vi "SMO.jsonRPC.SendAsyncRequest.vi"(7 "Notification":bool, 8 "error in (no error)":errorcluster, 9 "Parameters":variant, 10 "Method":string, 11 "SMO.jsonRPC in":refnum<class "SMO.jsonRPC.lvclass">) -> (0 "error out":errorcluster, 2 "id":i32, 3 "SMO.jsonRPC out":refnum<class "SMO.jsonRPC.lvclass">)   [LabVIEW 2013, in "SMO.jsonRPC.lvclass"]
uses:
  SMO.jsonRPC.lvclass
  Typedefs/Request--Cluster.ctl
  <vilib>/JKI/JKI JSON RPC Specification/Request/Request.lvclass
  <vilib>/JKI/JKI JSON RPC Specification/Response/Response.lvclass
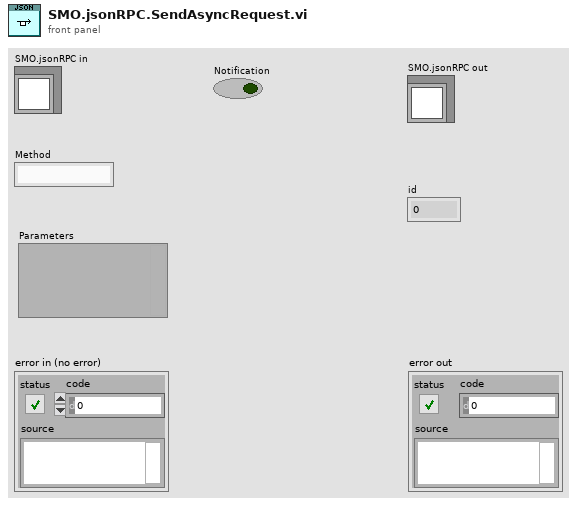
[diagram p1: front panel]
types:
  T1 = typedef "SMO.jsonRPC.lvclass/Request--Cluster.ctl" = cluster{"Request":refnum<class "Request.lvclass">, "reply queue":refnum<queue>, "Async?":bool}
  T2 = typedef "SMO.jsonRPC.lvclass/PrivateEvents--Cluster.ctl" = cluster{"Incoming Request":refnum<user-event>}
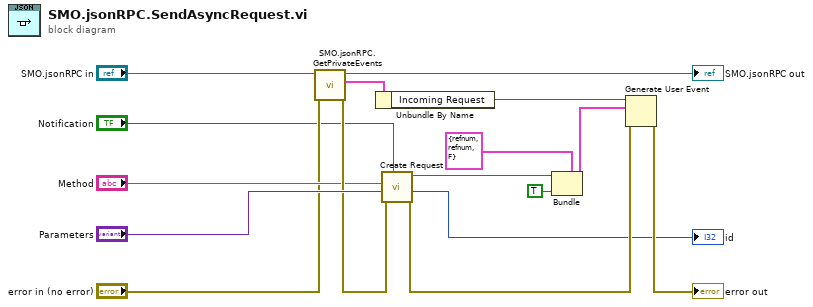
[diagram p0: block diagram]
diagram:
  n1 = call "SMO.jsonRPC.GetPrivateEvents.vi"("error in (no error)"="error in (no error)", "SMO.jsonRPC"="SMO.jsonRPC in") -> ("error out"=w14:errorcluster, "Private Events"=w7:T2, "SMO.jsonRPC out"=→"SMO.jsonRPC out":refnum<class "SMO.jsonRPC.lvclass">)  [unwired: 7 in]
  n2 = Unbundle By Name(w7) -> ("Incoming Request"=w6:refnum<user-event>)
  n3 = call <vilib>:"Create Request.vi"("Notification (F)"="Notification", "error in (no error)"=w14, "Parameters"="Parameters", "Method"="Method") -> ("error out"=w15:errorcluster, "id"=→"id":i32, "Request"=w12:refnum<class "Request.lvclass">)  [unwired: 4 in, 1 out]
  n4 = Bundle(cluster=T1 {"Request"=refnum, "reply queue"=refnum, "Async?"=FALSE} ("event data"), "Request"=w12, "Async?"=TRUE) -> (w9:T1)  [unwired: 1 in]
  n5 = Generate User Event(user event=w6, event data cluster=w9, error in=w15) -> (error out=→"error out":errorcluster)  [unwired: 1 in, 1 out]
